vi "escapeXML.vi"(10 "Input String":string) -> (2 "XML-escaped String":string)   [LabVIEW 2020, in "Caraya.lvlib" / "Test Report.JUnit.lvclass"]
uses:
  Test Report.JUnit.lvclass
  MsgSerializer.XML/MsgSerializer.XML.lvclass
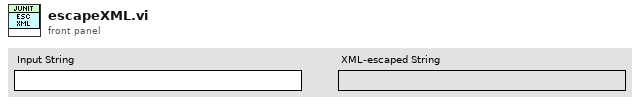
[diagram p1: front panel]
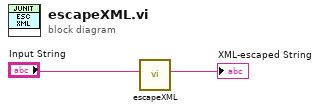
[diagram p0: block diagram]
diagram:
  n1 = call "escapeXML.vi"("Input String"="Input String") -> ("XML-escaped String"=→"XML-escaped String":string)  [unwired: 10 in]
